vi "Actor Core.vi"(8 "error in":errorcluster, 11 "ZM-HWM-hardware_manager in":refnum<class "ZM-HWM-hardware_manager.lvclass">) -> (0 "error out":errorcluster, 3 "Actor out":refnum<class "Actor.lvclass">)   [LabVIEW 2020, in "ZM-HWM-hardware_manager.lvlib" / "ZM-HWM-hardware_manager.lvclass"]
doc: "Actor Core override of the hardware manager. ZM-HWM-init registers for the stop event before Call Parent; ZM-HWM-helperAcquisition runs beside Call Parent. After Call Parent, ZM-HWM-stop ends the helper loop and ZM-HWM-close destroys the event. Error-handling plan: none yet; a helper-loop error goes to error out and the Last Ack, and stops the caller."
uses:
  ZM-HWM-hardware_manager.lvclass
  <vilib>/ActorFramework/Actor/Actor.lvclass
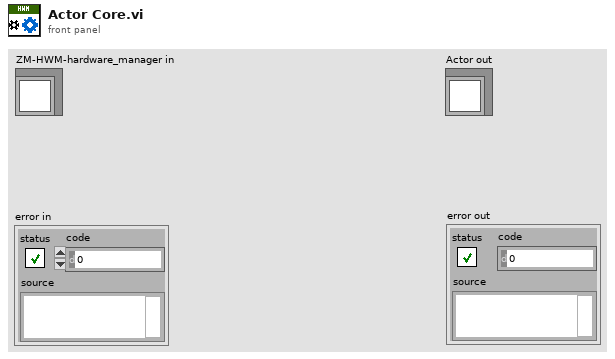
[diagram p1: front panel]
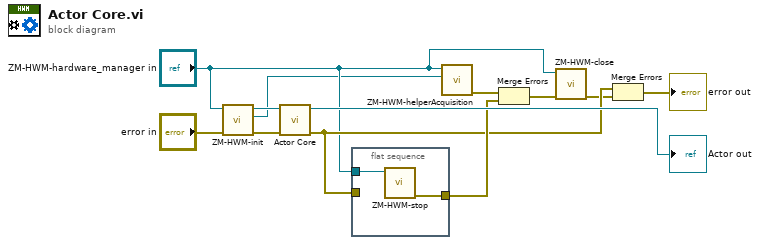
[diagram p0: block diagram]
diagram:
  n1 = call "ZM-HWM-init.vi"("error in"="error in", "ZM-HWM-hardware_manager in"="ZM-HWM-hardware_manager in") -> ("error out"=w2:errorcluster, "event registration refnum"=w1:refnum<event-registration>, "ZM-HWM-hardware_manager out"=w4:refnum<class "ZM-HWM-hardware_manager.lvclass">)  [unwired: 7 in]
  n2 = call-parent "Actor Core.vi"("error in"=w2, "Actor in"=w4) -> ("error out"=w8:errorcluster, "Actor out"=→"Actor out":refnum<class "Actor.lvclass">)  [unwired: 8 in]
  n3 = flat-sequence {
    tunnel: "ZM-HWM-hardware_manager in" -> [w14]
    tunnel: [w13] -> w9
    tunnel: w8 -> [_]
    frame #0 {
      n4 = call "ZM-HWM-stop.vi"("ZM-HWM-hardware_manager in"=w14) -> ("error out"=w13:errorcluster)  [unwired: 9 in, 1 out]
    }
  }
  n5 = call "ZM-HWM-helperAcquisition.vi"("event registration refnum"=w1, "ZM-HWM-hardware_manager in"="ZM-HWM-hardware_manager in") -> ("error out"=w11:errorcluster)  [unwired: 9 in]
  n6 = Merge Errors(w11, w9) -> (w10:errorcluster)
  n7 = call "ZM-HWM-close.vi"("error in (no error)"=w10, "ZM-HWM-hardware_manager in"="ZM-HWM-hardware_manager in") -> ("error out"=w7:errorcluster)  [unwired: 8 in, 1 out]
  n8 = Merge Errors(w8, w7) -> (→"error out":errorcluster)
